vi "Get All Case and Event Frames.vi"(8 "error in (no error)":errorcluster, 11 "JKI SM in":refnum<class "JKI SM.lvclass">) -> (0 "error out":errorcluster, 1 "Event Structure Visible?":bool, 2 "Frame Names":string[](array[string]), 3 "Frames[]":refnum<vi>[](array[refnum]), 4 "Visible Frame Index":i32, 5 "Visible Frame":refnum<vi>, 6 "Visible Frame Name":string, 7 "Num Event Frames":i32, 9 "Event Frame Index":i32)   [LabVIEW 2020]
uses:
  JKI State Machine API/source/JKI SM/JKI SM.lvclass
  JKI State Machine API/source/JKI SM/JKI SM.lvclass/JKI SM.ctl
  <userlib>/_OpenG.lib/string/string.llb/openg_string.lvlib
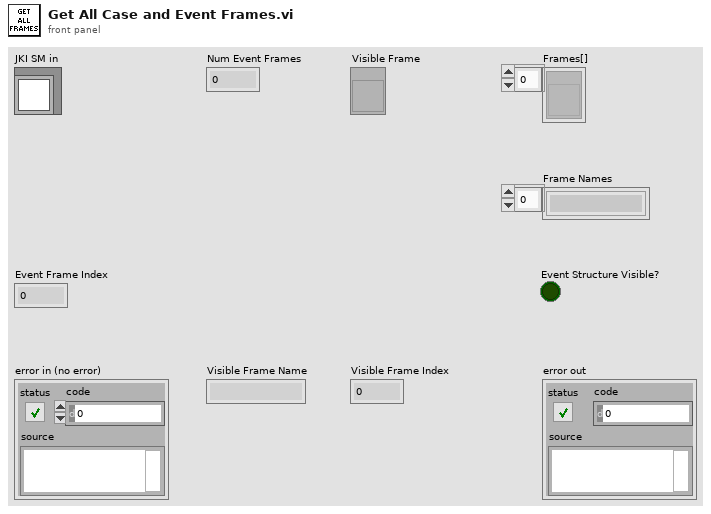
[diagram p1: front panel]
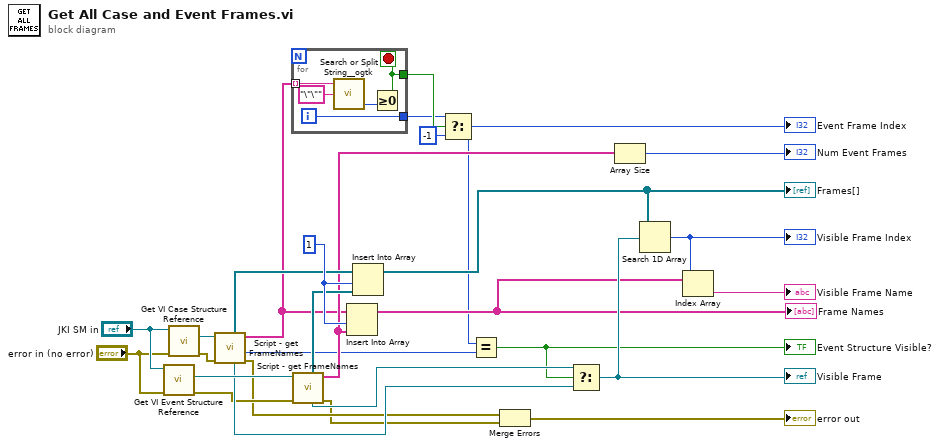
[diagram p0: block diagram]
diagram:
  w28 = 1 ("index")
  n1 = call "Get VI Event Structure Reference.vi"("error in (no error)"="error in (no error)", "JKI SM in"="JKI SM in") -> ("error out"=w7:errorcluster, "Event Structure ref"=w25:refnum<vi>)  [unwired: 7 in, 1 out]
  n2 = call "Get VI Case Structure Reference.vi"("error in (no error)"="error in (no error)", "JKI SM in"="JKI SM in") -> ("error out"=w8:errorcluster, "Case Structure ref"=w24:refnum<vi>)  [unwired: 7 in, 1 out]
  n3 = call "Script - get FrameNames.vi"("error in"=w8, "StructRef"=w24) -> ("error out"=w6:errorcluster, "Visible Frame Index"=w2:u32, "Frame Names"=w14:string[], "Visible Frame"=w22:refnum<vi>, "Frames[]"=w27:refnum<vi>[])  [unwired: 4 in, 1 out]
  n4 = for {
    tunnel: w14 -> [w33] mode=indexing
    tunnel: [w29] -> w13
    tunnel: [w30] -> w12
    i -> [w30]
    stop <- w29 stop-if-true
    n5 = call <userlib>:"Search or Split String__ogtk.vi"("search string/char (-)"="\"\"", "string"=w33) -> ("offset after match"=w31:i32)  [unwired: 1 in, 2 out]
    n6 = Greater Or Equal To 0?(x=w31) -> (x >= 0?=w29:bool)
  }
  n7 = call "Script - get FrameNames.vi"("error in"=w7, "StructRef"=w25) -> ("error out"=w5:errorcluster, "Frame Names"=w16:string[], "Visible Frame"=w23:refnum<vi>, "Frames[]"=w26:refnum<vi>[])  [unwired: 4 in, 2 out]
  n8 = Insert Into Array(array=w14, index=w28, new element=w16) -> (w18:string[])
  "Frame Names" <- w18
  n9 = Insert Into Array(array=w27, index=w28, new element=w26) -> (w21:refnum<vi>[])
  "Frames[]" <- w21
  n10 = Select(t=w12, s=w13, f=-1) -> (s? t:f=w3:i32)
  "Event Frame Index" <- w3
  n11 = Equal?(x=w3, y=w2) -> (x = y?=w1:bool)
  "Event Structure Visible?" <- w1
  n12 = Merge Errors(w6, w5) -> (→"error out":errorcluster)
  n13 = Select(t=w23, s=w1, f=w22) -> (s? t:f=w20:refnum<vi>)
  "Visible Frame" <- w20
  n14 = Array Size(array=w16) -> (size(s)=→"Num Event Frames":i32)
  n15 = Search 1D Array(1D array=w21, element=w20) -> (index of element=w19:i32)  [unwired: 1 in]
  "Visible Frame Index" <- w19
  n16 = Index Array(array=w18, index=w19) -> (element=→"Visible Frame Name":string)
